vi "Groups for Channels.vi"(8 "error in (no error)":errorcluster, 10 "Channels":string[](array[string]), 11 "VolatusAPI in":refnum<class "VolatusAPI.lvclass">) -> (0 "error out":errorcluster, 1 "Channels per Group":cluster{cluster{"Index":i32, "Name":string}[]}[](array[cluster]), 2 "Groups":string[](array[string]), 3 "VolatusAPI out":refnum<class "VolatusAPI.lvclass">)   [LabVIEW 2020, in "Volatus.lvlib" / "VolatusAPI.lvclass"]
uses:
  VolatusAPI.lvclass
  <vilib>/Utility/miscctls.llb/LVMapReplaceAction.ctl
  VolatusAPI.lvclass/VolatusAPI.ctl
  lv-vecto/Vecto/Group/Group.lvclass
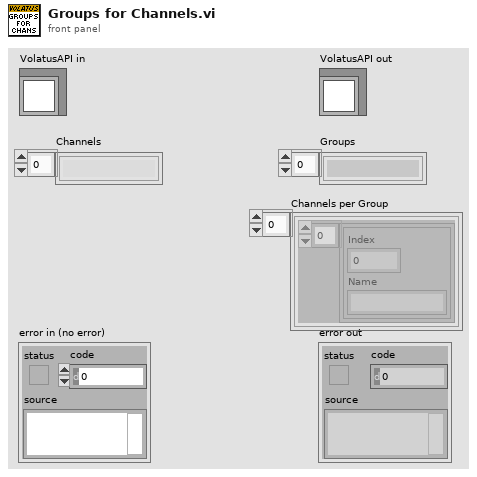
[diagram p1: front panel]
types:
  T1 = map{string, cluster{"Index":i32, "String":string}[]}
  T2 = typedef "LVMapReplaceAction.ctl" = enum32{"Modify Entry only if found", "Add or Modify Entry", "Delete Entry"}
  T3 = typedef "VectoConfig.lvlib/Channel Info.ctl" = cluster{"Name":string, "Group":string, "Owning Node":string, "Owning Task":string, "Resource":string}
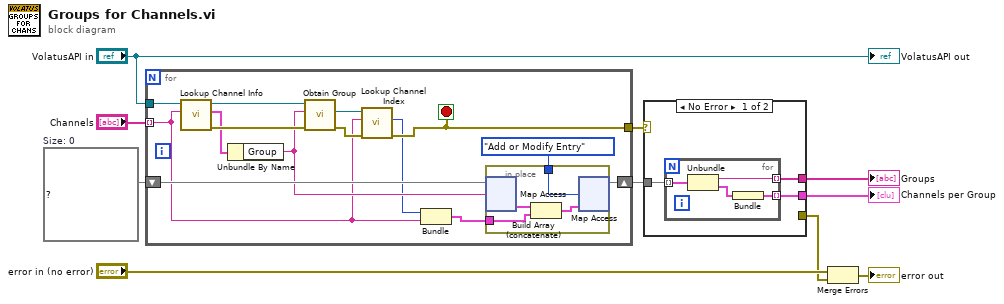
[diagram p0: block diagram]
diagram:
  w6 = T1 {}  # Size: 0
  n1 = for {
    tunnel: "Channels" -> [w13] mode=indexing
    tunnel: "VolatusAPI in" -> [w22]
    shift-right: [w18] -> w5
    shift-left: w6 -> [w20]
    tunnel: [w24] -> w4
    stop <- w24 stop-if-true
    n2 = call "Lookup Channel Info.vi"("Channel Name"=w13, "VolatusAPI in"=w22) -> ("error out"=w23:errorcluster, "Channel Info"=w21:T3, "VolatusAPI out"=w17:refnum<class "VolatusAPI.lvclass">)  [unwired: 6 in, 1 out]
    n3 = Unbundle By Name(w21) -> ("Group"=w16:string)
    n4 = call "Obtain Group.vi"("error in (no error)"=w23, "Group Name"=w16, "VolatusAPI in"=w17) -> ("error out"=w14:errorcluster, "Group"=w15:refnum<class "Group.lvclass">)  [unwired: 6 in, 1 out]
    n5 = call "Lookup Channel Index.vi"("error in (no error)"=w14, "Channel Name"=w13, "Group in"=w15) -> ("error out"=w24:errorcluster, "Index"=w11:i32)  [unwired: 6 in, 1 out]
    n6 = Bundle("Index"=w11, "String"=w13) -> (w12:cluster{"Index":i32, "String":string})  [unwired: 1 in]
    n7 = in-place {
      in-place-border: w12 -> [w27]
      in-place-border: LVMapReplaceAction."Add or Modify Entry" ("action") -> [w25]
      n8 = in-place-map #1(w20, w16) -> (w28:cluster{"Index":i32, "String":string}[])  [unwired: 1 in, 1 out]
      n9 = Build Array (concatenate)(w28, w27) -> (w26:cluster{"Index":i32, "String":string}[])
      n10 = in-place-map #1(w26, w25) -> (w18:T1)  [unwired: 2 out]
    }
  }
  n11 = case shown="No Error" w4 {
    selector: w4 -> [_ w36]
    tunnel: w5 -> [w31 _]
    tunnel: [w30 _] -> w1
    tunnel: [w29 _] -> w3
    tunnel: [_ w36] -> w2
    frame No Error {
      n12 = for {
        tunnel: w31 -> [w35] mode=indexing
        tunnel: [w33] -> w30 mode=indexing
        tunnel: [w32] -> w29 mode=indexing
        n13 = Unbundle(w35) -> (w32:string, w34:cluster{"Index":i32, "String":string}[])
        n14 = Bundle(w34) -> (w33:cluster{cluster{"Index":i32, "String":string}[]})  [unwired: 1 in]
      }
    }
    frame Error {
    }
  }
  "Groups" <- w3
  "Channels per Group" <- w1
  n15 = Merge Errors("error in (no error)", w2) -> (→"error out":errorcluster)
  "VolatusAPI out" <- "VolatusAPI in"
